vi "Save For Previous.vi"() -> ()   [LabVIEW 2020]
doc: "Dev helper: saves every VI listed in the items file (one path per line) for a previous LabVIEW version, in place (Save.For Previous to its own path). Returns the error code, source and Save for previous warnings per item, in list order. The VIs stay in memory in the current version: close them without saving afterwards."
panel:
  out "error out":errorcluster
  out "warnings":string[](array[string])
  out "sources":string[](array[string])
  out "codes":i32[](array[numeric])
  in  "version":string="20.0"
  in  "items file":path
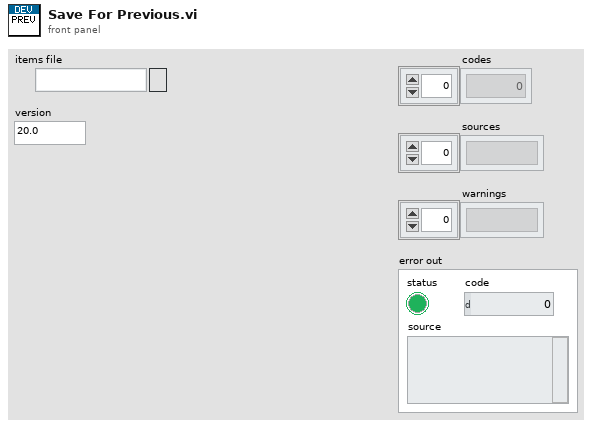
[diagram p1: front panel]
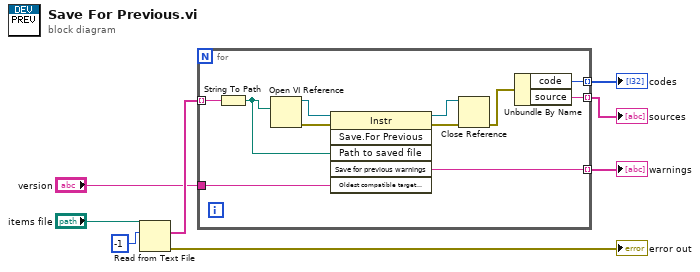
[diagram p0: block diagram]
diagram:
  n1 = Read from Text File(file (use dialog)="items file", count=-1) -> (text=w6:string[], error out=→"error out":errorcluster)  [unwired: 2 in, 2 out]
  n2 = for {
    tunnel: w6 -> [w19] mode=indexing
    tunnel: "version" -> [w15]
    tunnel: [w11] -> w4 mode=indexing
    tunnel: [w10] -> w2 mode=indexing
    tunnel: [w9] -> w3 mode=indexing
    n3 = String To Path(string=w19) -> (path=w16:path)
    n4 = Open VI Reference(vi path=w16) -> (vi reference=w18:refnum<vi>, error out=w17:errorcluster)  [unwired: 5 in]
    n5 = invoke class="Instr" method="Save.For Previous"(reference=w18, error in=w17, "Path to saved file"=w16, "Oldest compatible target version"=w15) -> (reference out=w14:refnum<vi>, error out=w13:errorcluster, "Save for previous warnings"=w10:string)  [unwired: 2 in, 3 out]
    n6 = Close Reference(reference=w14, error in (no error)=w13) -> (error out=w12:errorcluster)
    n7 = Unbundle By Name(w12) -> ("code"=w11:i32, "source"=w9:string)
  }
  "codes" <- w4
  "sources" <- w3
  "warnings" <- w2
